vi "MPExxx Set Register.vi"(2 "error in (no error)":errorcluster {"code" format="%.0x"}, 3 "Value":u8, 4 "Standard Commands":u8(ring) items=["Clear Interface", "Event Status Enable", "Recall", "Save", "Service Request Enable"], 5 "VISA session":refnum<visa-resource-name>) -> (0 "error out":errorcluster {"code" format="%.0x"}, 1 "dup VISA session":refnum<visa-resource-name>)   [LabVIEW 2012]
doc: "Sets the power supply's register values."
panel:
  # "MAGNA-POWER"
  # "Electronics"
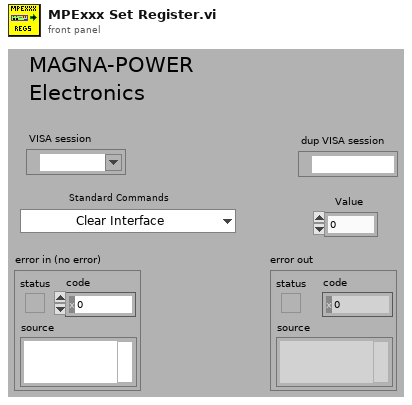
[diagram p1: front panel]
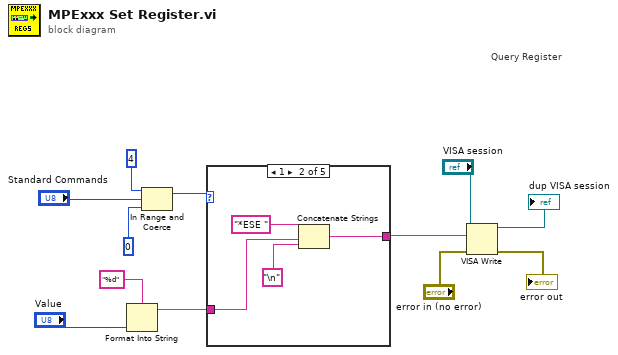
[diagram p0: block diagram]
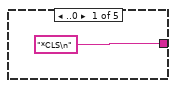
[diagram p2: hidden frame]
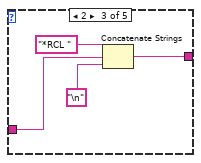
[diagram p3: hidden frame]
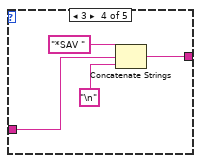
[diagram p4: hidden frame]
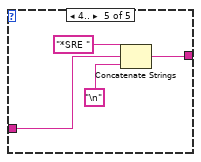
[diagram p5: hidden frame]
diagram:
  # "Query Register"
  n1 = Format Into String(format string="%d" ("Format String"), "Value") -> (resulting string=w1:string)  [unwired: 2 in, 1 out]
  n2 = In Range and Coerce(upper limit=4, x="Standard Commands", lower limit=0) -> (coerced(x)=w5:i32)  [unwired: 1 out]
  n3 = case shown="1" w5 {
    tunnel: ["*CLS\n" w15 w19 w23 w27] -> w10
    tunnel: w1 -> [_ w14 w18 w22 w26]
    frame ..0 {
    }
    frame 1 {
      n4 = Concatenate Strings("*ESE ", w14, "\n") -> (w15:string)
    }
    frame 2 {
      n5 = Concatenate Strings("*RCL ", w18, "\n") -> (w19:string)
    }
    frame 3 {
      n6 = Concatenate Strings("*SAV ", w22, "\n") -> (w23:string)
    }
    frame 4.. {
      n7 = Concatenate Strings("*SRE ", w26, "\n") -> (w27:string)
    }
  }
  n8 = VISA Write(VISA resource name="VISA session", write buffer=w10, error in (no error)="error in (no error)") -> (VISA resource name out=→"dup VISA session":refnum<visa-resource-name>, error out=→"error out":errorcluster)  [unwired: 1 out]
